vi "Panel.vi"(11 "DeviceArrayPanel in":refnum<class "DeviceArrayPanel.lvclass">) -> ()   [LabVIEW 2020, in "PicoG-App.lvlib" / "DeviceArrayPanel.lvclass"]
uses:
  DeviceArrayPanel.lvclass
  C:/Program Files (x86)/National Instruments/LabVIEW 2020/vi.lib/IlluminatedG/IG OOPanel/OOPanel/Panel/Panel.lvclass
  <vilib>/IlluminatedG/IG OOPanel/OOPanel/Panel/Basic UI State.ctl
  DeviceArrayPanel.lvclass/DeviceArrayPanel.ctl
  Device/Get ID.vi
  Device/Get Alias.vi
  Device/Get Platform Name.vi
  Device/Get Board.vi
  Device/Get Version String.vi
  Device/Get Picture.vi
  <vilib>/IlluminatedG/IG OOPanel/OOPanel/Panel/Panel.lvclass
  <vilib>/IlluminatedG/IG OOPanel/OOPanel/OOPanel.lvlib
  Device/Device.lvclass
panel:
  out "Picture":picture
  out "ID":string="E6605838830B8539"
  out "Version String":string="0.0.3"
  out "Board":string="pico"
  out "Platform Name":string="RP2040"
  out "Alias":string="NomadPico"
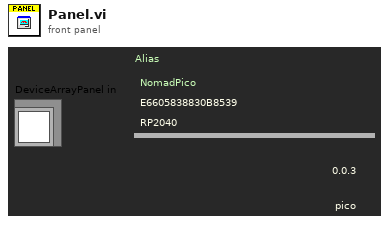
[diagram p1: front panel]
types:
  T1 = typedef "OOPanel.lvlib/Panel.lvclass/Basic UI State.ctl" = enum16{"Init", "Run", "Close"}
  T2 = typedef "PicoG-App.lvlib/DeviceArrayPanel.lvclass/Inbound Events.ctl" = cluster{"Set Highlighted":refnum<user-event>, "Refresh":refnum<user-event>}
  T3 = typedef "OOPanel.lvlib/Panel.lvclass/Panel Events.ctl" = cluster{"Visbility":refnum<user-event>, "Close":refnum<user-event>}
  T4 = typedef "PicoG-App.lvlib/DeviceArrayPanel.lvclass/Ref Data.ctl" = cluster{"Device":refnum<class "Device.lvclass">}
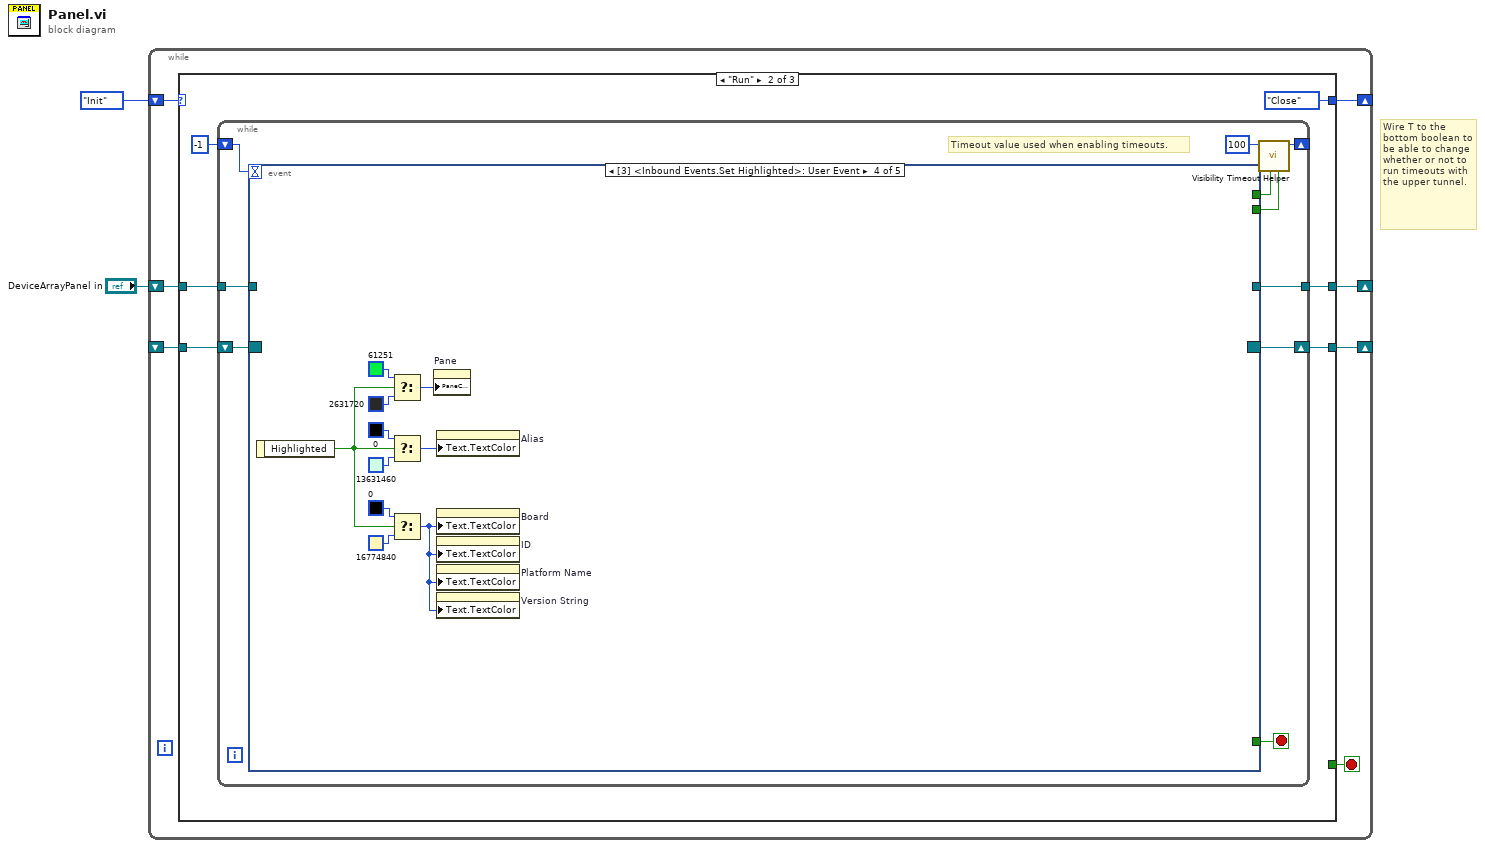
[diagram p0: block diagram]
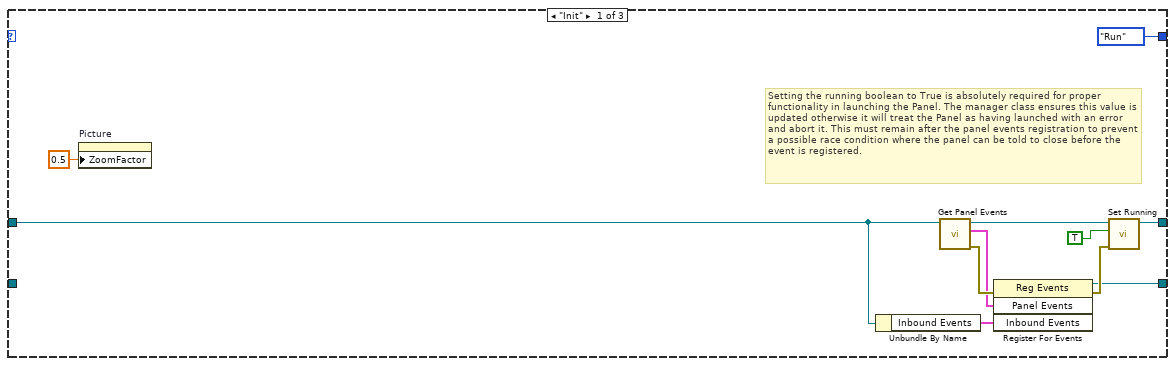
[diagram p2: hidden frame]
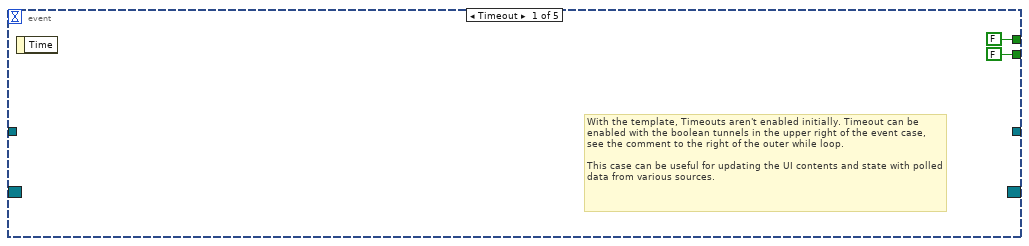
[diagram p3: hidden frame]
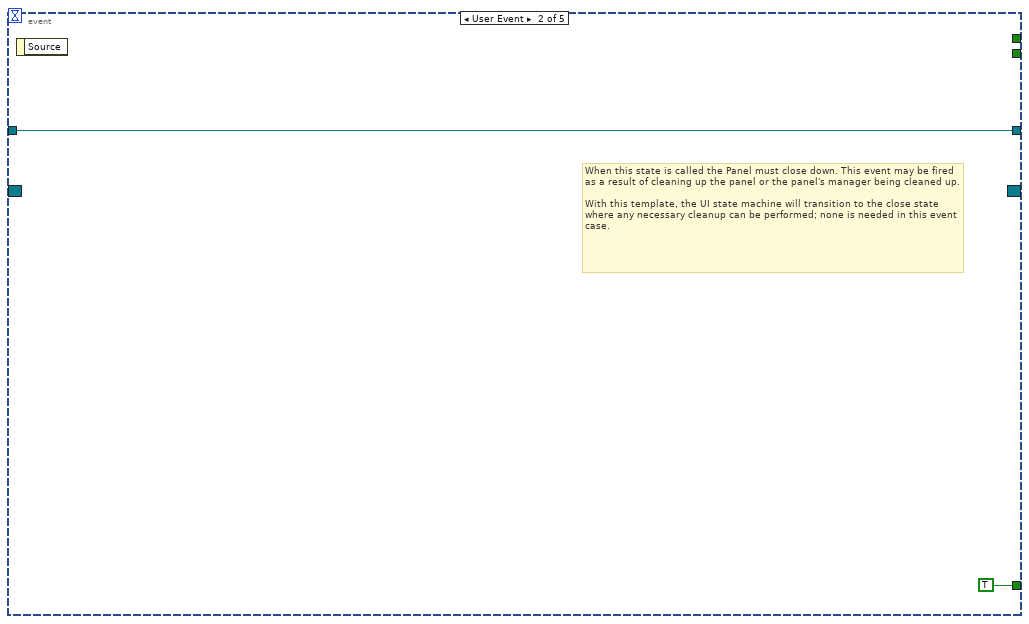
[diagram p4: hidden frame]
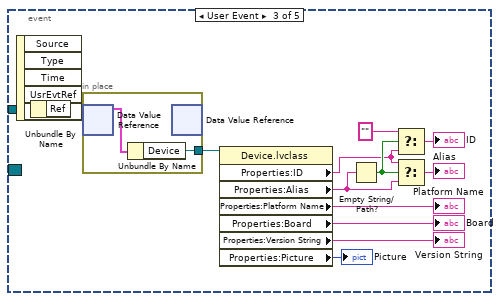
[diagram p5: hidden frame]
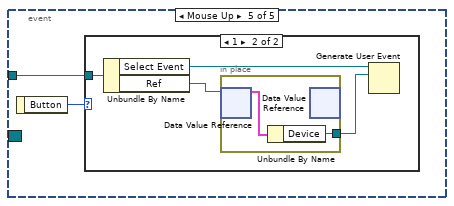
[diagram p6: hidden frame]
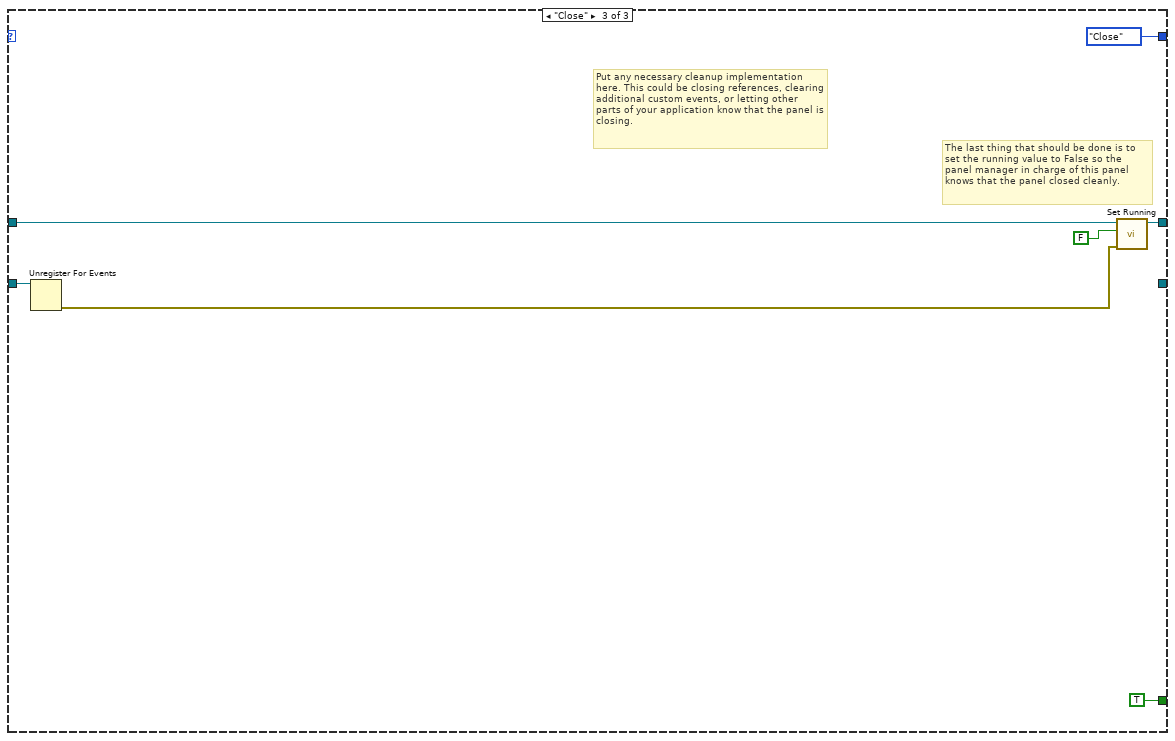
[diagram p8: hidden frame]
diagram:
  # "Wire T to the bottom boolean to be able to change whether or not to run timeouts with the upper tunnel."
  n1 = while {
    shift-right: [w8] -> _
    shift-left: _ -> [w9]
    shift-right: [w6] -> _
    shift-left: Basic_UI_State."Init" ("Basic UI State") -> [w7]
    shift-right: [w4] -> _
    shift-left: "DeviceArrayPanel in" -> [w3]
    stop <- w5 stop-if-true
    n2 = case shown="\"Run\"" w7 {
      tunnel: w9 -> [_ w26 w76]
      tunnel: [w14 w24 _] -> w8
      tunnel: [Basic_UI_State."Run" ("Basic UI State") Basic_UI_State."Close" ("Basic UI State") Basic_UI_State."Close" ("Basic UI State")] -> w6
      tunnel: [_ _ TRUE] -> w5
      tunnel: [w13 w21 w74] -> w4
      tunnel: w3 -> [w12 w22 w75]
      frame "Init" {
        # "Setting the running boolean to True is absolutely required for proper functionality in launching the Panel. The manager class ensures this value is updated otherwise it will treat the Panel as having launched with an error and abort it. This must remain after the panel events registration to prevent a possible race condition where the panel can be told to close before the event is registered."
        n3 = property on="Picture" class="Pict"("ZoomFactor"=sgl 0.5 ("Zoom Factor")) -> ()  [unwired: 2 in, 2 out]
        n4 = Unbundle By Name(w12) -> ("Inbound Events"=w11:T2)
        n5 = call <vilib>:"Get Panel Events.vi"("Panel in"=w12) -> ("error out"=w20:errorcluster, "Panel Events"=w16:T3, "Panel out"=w17:refnum<class "DeviceArrayPanel.lvclass">)  [unwired: 8 in]
        n6 = register-events(error in=w20, w16, w11) -> (reference out=w14:refnum<event-registration>, error out=w18:errorcluster)  [unwired: 1 in]
        n7 = call <vilib>:"Set Running.vi"("error in (no error)"=w18, "Running"=TRUE, "Panel in"=w17) -> ("Panel out"=w13:refnum<class "DeviceArrayPanel.lvclass">)  [unwired: 7 in, 1 out]
      }
      frame "Run" {
        n8 = while {
          shift-right: [w32] -> w24
          shift-left: w26 -> [w33]
          shift-right: [w35] -> _
          shift-left: -1 ("Timeout") -> [w34]
          tunnel: w22 -> [w28]
          tunnel: [w27] -> w21
          stop <- w29 stop-if-true
          # "Timeout value used when enabling timeouts."
          n9 = event shown="[3] <Inbound Events.Set Highlighted>: User Event" {
            selector: w33 -> [_ _ _ _ _]
            dyn-events: [_ _ _ _ _] -> w32
            timeout: w34 -> [_ _ _ _ _]
            tunnel: [FALSE _ _ _ _] -> w31
            tunnel: [FALSE _ _ _ _] -> w30
            tunnel: [_ TRUE _ _ _] -> w29
            tunnel: w28 -> [_ w39 w52 _ w67]
            tunnel: [_ w39 _ _ _] -> w27
            event Timeout {
              # "With the template, Timeouts aren't enabled initially. Timeout can be enabled with the boolean tunnels in the upper right of the event case, see the comment to the right of the outer while loop.\n\nThis case can be useful for updating the UI contents and state with polled data from various sources."
              n10 = event-data() -> ()  [unwired: 1 in, 1 out]
            }
            event User Event {
              # "When this state is called the Panel must close down. This event may be fired as a result of cleaning up the panel or the panel's manager being cleaned up.\n\nWith this template, the UI state machine will transition to the close state where any necessary cleanup can be performed; none is needed in this event case."
              n11 = event-data() -> ()  [unwired: 1 in, 1 out]
            }
            event User Event {
              n12 = event-data() -> ()  [unwired: 1 in, 5 out]
              n13 = Unbundle By Name(w52) -> ("Ref"=w53:refnum<data-value>)
              n14 = in-place {
                in-place-border: [w54] -> w51
                n15 = in-place-dvr #1(w53) -> (w55:T4)  [unwired: 1 out]
                n16 = Unbundle By Name(w55) -> ("Device"=w54:refnum<class "Device.lvclass">)
                n17 = in-place-dvr #1() -> ()  [unwired: 1 in, 2 out]
              }
              n18 = property class="Device.lvclass"(reference=w51) -> ("Properties:ID"=w44:string, "Properties:Alias"=w50:string, "Properties:Platform Name"=→"Platform Name":string, "Properties:Board"=→"Board":string, "Properties:Version String"=→"Version String":string, "Properties:Picture"=→"Picture":picture)  [unwired: 1 in, 2 out]
              n19 = Empty String/Path?(string/path=w50) -> (empty?=w45:bool)
              n20 = Select(t="", s=w45, f=w44) -> (s? t:f=→"ID":string)
              n21 = Select(t=w44, s=w45, f=w50) -> (s? t:f=→"Alias":string)
            }
            event User Event {
              n22 = event-data() -> ("Highlighted"=w57:bool)  [unwired: 1 in]
              n23 = Select(t=u32 61251, s=w57, f=u32 2631720) -> (s? t:f=w63:u32)
              n24 = Select(t=u32 0, s=w57, f=u32 13631460) -> (s? t:f=w60:u32)
              n25 = Select(t=u32 0, s=w57, f=u32 16774840) -> (s? t:f=w56:u32)
              n26 = property on="Pane" class="Pane"("PaneColor"=w63) -> ()  [unwired: 2 in, 2 out]
              n27 = property on="Alias" class="Str"("Text.TextColor"=w60) -> ()  [unwired: 2 in, 2 out]
              n28 = property on="Board" class="Str"("Text.TextColor"=w56) -> ()  [unwired: 2 in, 2 out]
              n29 = property on="ID" class="Str"("Text.TextColor"=w56) -> ()  [unwired: 2 in, 2 out]
              n30 = property on="Platform Name" class="Str"("Text.TextColor"=w56) -> ()  [unwired: 2 in, 2 out]
              n31 = property on="Version String" class="Str"("Text.TextColor"=w56) -> ()  [unwired: 2 in, 2 out]
            }
            event Mouse Up {
              n32 = event-data() -> ("Button"=w66:u16)  [unwired: 1 in]
              n33 = case shown="1" w66 {
                tunnel: w67 -> [_ w70]
                frame Default {
                }
                frame 1 {
                  n34 = Unbundle By Name(w70) -> ("Select Event"=w69:refnum<user-event>, "Ref"=w71:refnum<data-value>)
                  n35 = in-place {
                    in-place-border: [w72] -> w68
                    n36 = in-place-dvr #2(w71) -> (w73:T4)  [unwired: 1 out]
                    n37 = Unbundle By Name(w73) -> ("Device"=w72:refnum<class "Device.lvclass">)
                    n38 = in-place-dvr #2() -> ()  [unwired: 1 in, 2 out]
                  }
                  n39 = Generate User Event(user event=w69, event data cluster=w68) -> ()  [unwired: 2 in, 2 out]
                }
              }
            }
          }
          n40 = call <vilib>:"Visibility Timeout Helper.vi"("Update?"=w30, "Use Timeout?"=w31, "Visible Timeout mS"=100) -> ("Timeout"=w35:i32)  [unwired: 8 in]
        }
      }
      frame "Close" {
        # "Put any necessary cleanup implementation here. This could be closing references, clearing additional custom events, or letting other parts of your application know that the panel is closing."
        # "The last thing that should be done is to set the running value to False so the panel manager in charge of this panel knows that the panel closed cleanly."
        n41 = Unregister For Events(event registration refnum=w76) -> (error out=w78:errorcluster)  [unwired: 1 in]
        n42 = call <vilib>:"Set Running.vi"("error in (no error)"=w78, "Running"=FALSE, "Panel in"=w75) -> ("Panel out"=w74:refnum<class "DeviceArrayPanel.lvclass">)  [unwired: 7 in, 1 out]
      }
    }
  }
